vi "Over Voltage_test.vi"(8 "error in (no error)":errorcluster) -> (0 "error out":errorcluster)   [LabVIEW 2025]
uses:
  SubVIs/All test cluster.ctl
  SubVIs/All_enum_ctl.ctl
  SubVIs/Arduino_lamps.ctl
  SubVIs/Lamps_global.vi
  <vilib>/Utility/file.llb/Write Delimited Spreadsheet (string).vi
  <instrlib>/BK Precision 9200 Series/BK Precision 9200 Series.lvlib
  <instrlib>/Keithley 2260B/Keithley 2260B.lvlib
panel:
  in  "ESP PORT":refnum<visa-resource-name>
  out "Connected? 2":bool caption="Long Blank Button"
  out "Tick Time(s)":dbl
  out "Status":string
  in  "POWER SUPPLY":bool caption="Blank Button"
  out "Text name":string
  in  "COM PORT:":refnum<visa-resource-name>
  in  "Start/Stop":bool caption="Slide Switch"
  in  "File Path:":path
  in  "FILENAME":string
  out "Table":string[][](table)
  out "Connected?":bool caption="Long Blank Button"
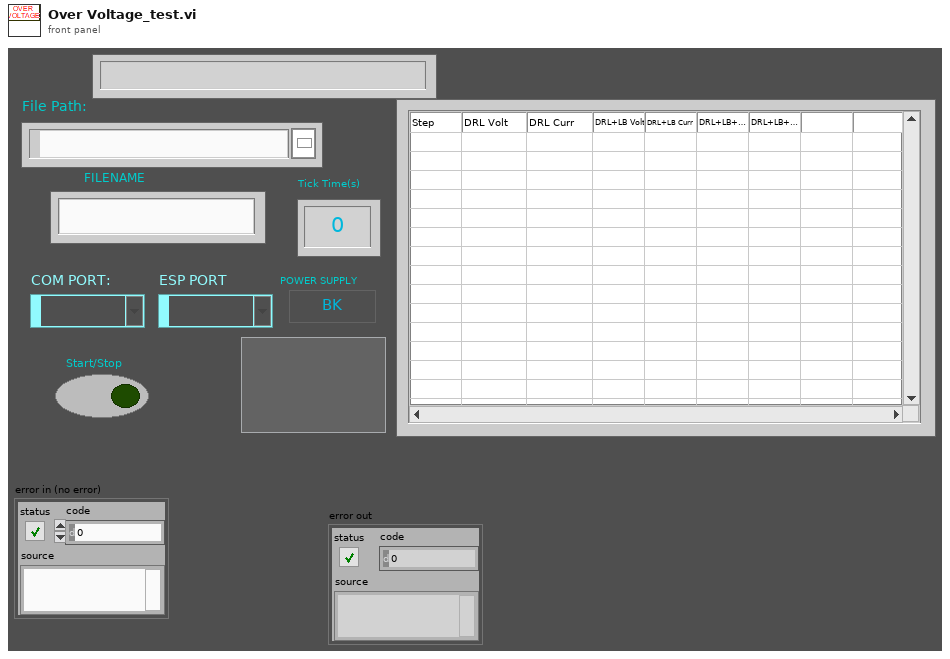
[diagram p1: front panel]
types:
  T1 = enum32{"Invalid", "Standard", "Closed", "Hidden", "Minimized", "Maximized"}
  T2 = typedef "All_enum_ctl.ctl" = enum16{"Init", "Poll", "Connect_esp32", "Connect", "check_start", "Start", "Set_Voltage", "On_relay", "Read_Voltage", "Off_Relay", "Next_Relay", "Next_Step", "Stop", "Store", "Error", "Exit"}
  T3 = typedef "All test cluster.ctl" = cluster{"FilePath":path, "Test Status":bool, "Start Volt":dbl, "End Volt":dbl, "Present Step":dbl, "Present Time(s)":dbl, "End Time":dbl, "Table":string[], "Intensity":string, "BK/Keith":bool, "COM":refnum<visa-resource-name>, "Next state":T2, "Step no.":dbl, "Start ms":u32, "ESP_COM":refnum<visa-resource-name>, "Relay_no":dbl, "Datas":string[]}
  T4 = typedef "Arduino_lamps.ctl" = enum16{"Init", "Poll", "Read", "Write", "Exit"}
  T5 = cluster{"Baud Rate":u32, "Parity":u16, "Data Bits":u16, "Stop Bits":u16, "Flow Control":u16}
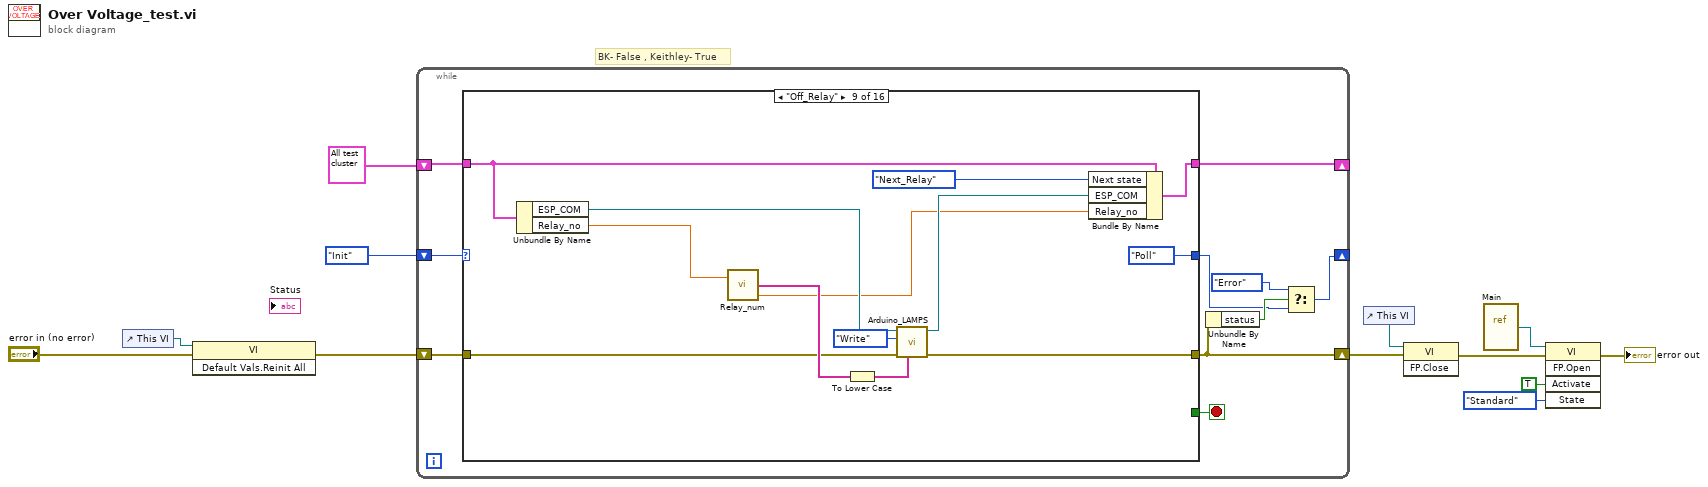
[diagram p0: block diagram]
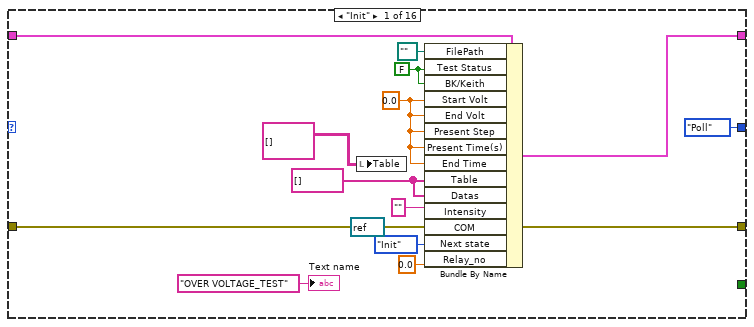
[diagram p2: hidden frame]
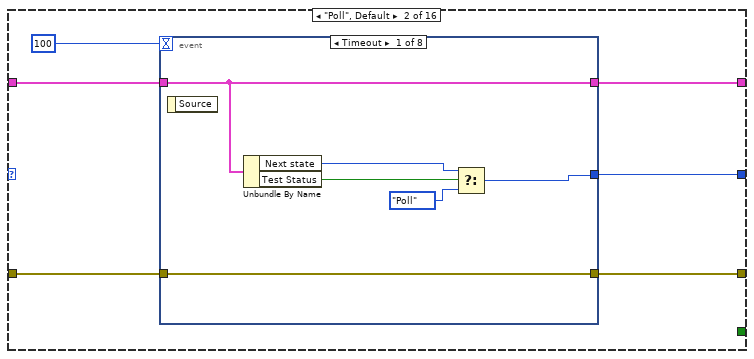
[diagram p3: hidden frame]
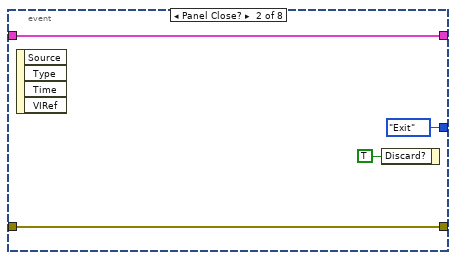
[diagram p4: hidden frame]
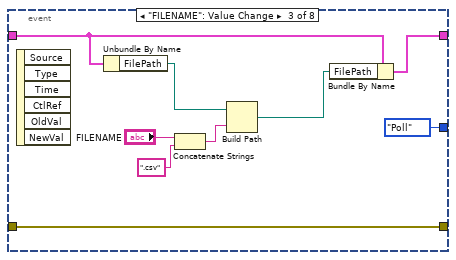
[diagram p5: hidden frame]
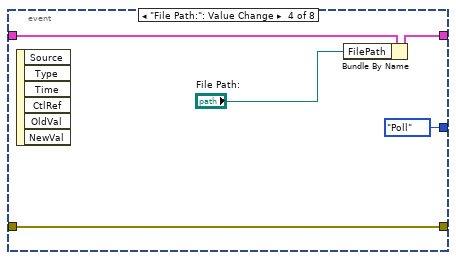
[diagram p6: hidden frame]
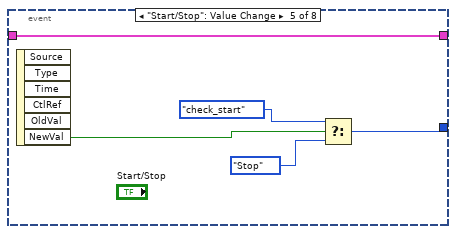
[diagram p7: hidden frame]
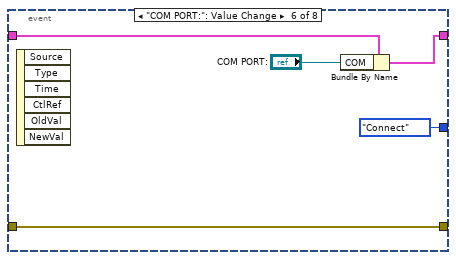
[diagram p8: hidden frame]
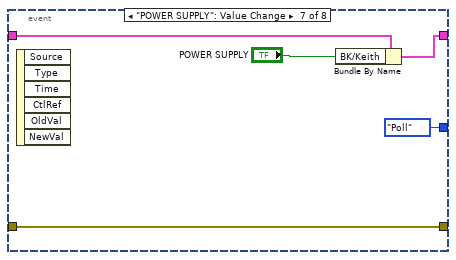
[diagram p9: hidden frame]
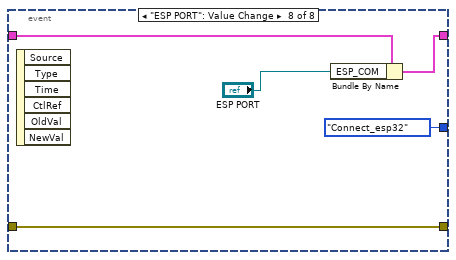
[diagram p10: hidden frame]
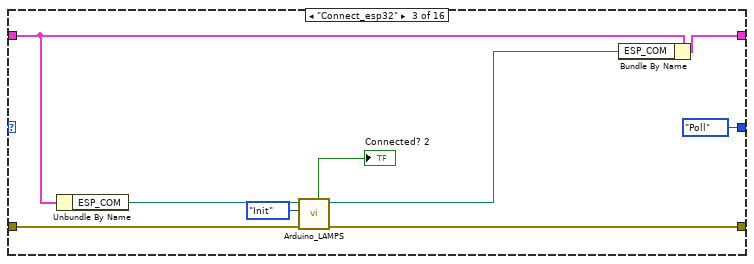
[diagram p11: hidden frame]
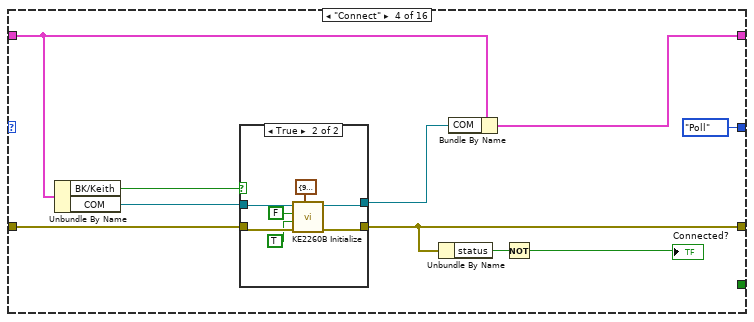
[diagram p12: hidden frame]
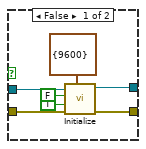
[diagram p13: hidden frame]
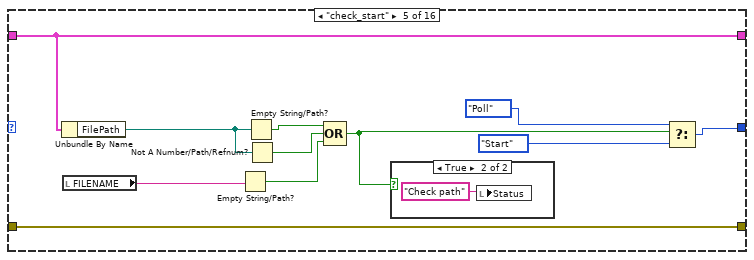
[diagram p14: hidden frame]
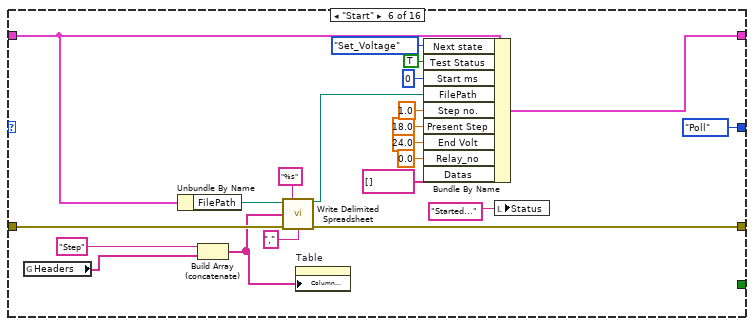
[diagram p16: hidden frame]
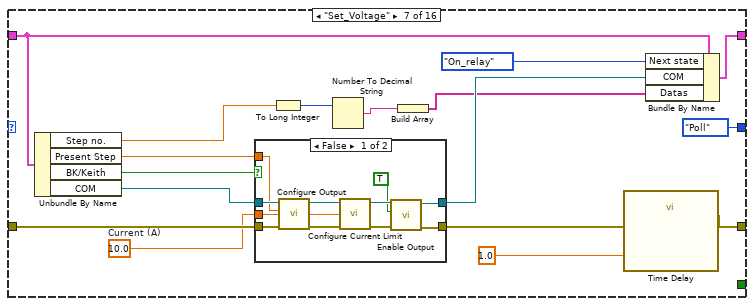
[diagram p17: hidden frame]
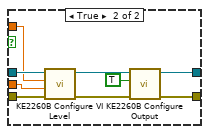
[diagram p18: hidden frame]
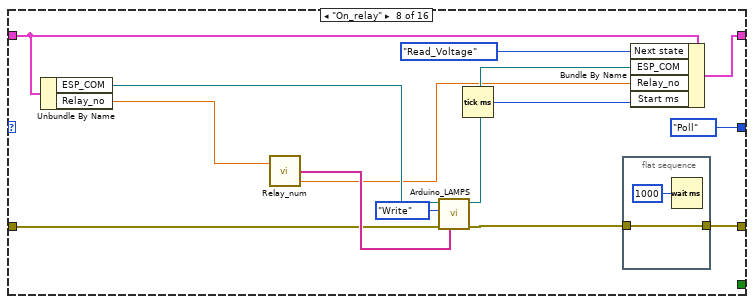
[diagram p19: hidden frame]
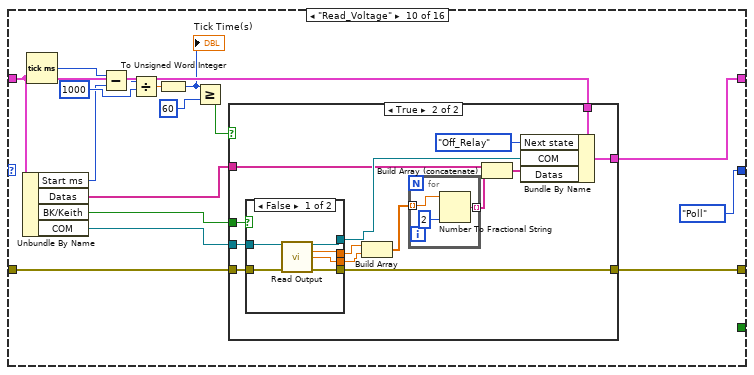
[diagram p20: hidden frame]
diagram:
  # "BK- False , Keithley- True"
  n1 = control-ref of="This VI"() -> (w12:refnum<vi>)
  n2 = invoke class="VI" method="Default Vals.Reinit All"(reference=w12, error in="error in (no error)") -> (error out=w10:errorcluster)  [unwired: 1 in, 2 out]
  n3 = while {
    shift-right: [w21] -> _
    shift-left: T3 {"FilePath"=path "", "Test Status"=FALSE, "Start Volt"=0.0, "End Volt"=0.0, "Present Step"=0.0, "Present Time(s)"=0.0, "End Time"=0.0, "Table"=[], "Intensity"="", "BK/Keith"=FALSE, "COM"="", "Next state"=enum."Init", "Step no."=0.0, "Start ms"=0, "ESP_COM"="", "Relay_no"=0.0, "Datas"=[]} -> [w20]
    shift-right: [w17] -> w2
    shift-left: w10 -> [w19]
    shift-right: [w13] -> _
    shift-left: All_enum_ctl."Init" -> [w22]
    stop <- w18 stop-if-true
    n4 = case shown="\"Off_Relay\"" w22 {
      tunnel: [w34 w39 w88 w97 w129 w151 w168 w192 w208 w229 w277 w314 w328 w342 w359 w379] -> w21
      tunnel: w20 -> [w36 w40 w91 w101 w129 w146 w167 w191 w207 w233 w278 w317 w323 w343 w362 w379]
      tunnel: w19 -> [w35 w42 w94 w105 w130 w148 w169 w195 w211 w234 w275 w318 w324 w347 w366 w384]
      tunnel: [w35 w41 w93 w100 w130 w147 w158 w194 w210 w232 w275 w311 w321 w347 w364 w380] -> w17
      tunnel: [All_enum_ctl."Poll" w37 All_enum_ctl."Poll" All_enum_ctl."Poll" w121 All_enum_ctl."Poll" All_enum_ctl."Poll" All_enum_ctl."Poll" All_enum_ctl."Poll" All_enum_ctl."Poll" All_enum_ctl."Poll" All_enum_ctl."Poll" All_enum_ctl."Poll" All_enum_ctl."Poll" All_enum_ctl."Poll" All_enum_ctl."Exit"] -> w14
      tunnel: [_ _ _ _ _ _ _ _ _ _ _ _ _ _ _ TRUE] -> w18
      frame "Init" {
        w24 = string[] [] ("Table")
        w32 = 0.0 ("Start Volt")
        w30 = FALSE ("Test Status")
        n5 = local write "Table"(string[][] [] ("Table")) -> ()
        n6 = Bundle By Name(cluster=w36, "FilePath"=path "", "Test Status"=w30, "BK/Keith"=w30, "Start Volt"=w32, "End Volt"=w32, "Present Step"=w32, "Present Time(s)"=w32, "End Time"=w32, "Table"=w24, "Datas"=w24, "Intensity"="", "COM"=refnum<visa-resource-name> refnum, "Next state"=All_enum_ctl."Init" ("Last state"), "Relay_no"=0.0) -> (w34:T3)
        "Text name" <- "OVER VOLTAGE_TEST" ("Text name")
      }
      frame "Poll", Default {
        n7 = event shown="[0] Timeout" {
          selector: _ -> [_ _ _ _ _ _ _ _]
          dyn-events: _ -> [_ _ _ _ _ _ _ _]
          timeout: 100 -> [_ _ _ _ _ _ _ _]
          tunnel: w42 -> [w48 w49 w61 w64 _ w72 w77 w82]
          tunnel: [w48 w49 w61 w64 _ w72 w77 w82] -> w41
          tunnel: w40 -> [w47 w50 w59 w66 w70 w76 w81 w85]
          tunnel: [w47 w50 w55 w63 w70 w75 w80 w86] -> w39
          tunnel: [w43 All_enum_ctl."Exit" ("f") All_enum_ctl."Poll" All_enum_ctl."Poll" w67 All_enum_ctl."Connect" ("f") All_enum_ctl."Poll" ("f") All_enum_ctl."Connect_esp32" ("f")] -> w37
          event Timeout {
            n8 = event-data() -> ()  [unwired: 1 in, 1 out]
            n9 = Unbundle By Name(w47) -> ("Next state"=w44:T2, "Test Status"=w46:bool)
            n10 = Select(t=w44, s=w46, f=All_enum_ctl."Poll") -> (s? t:f=w43:T2)
          }
          event Panel Close? {
            n11 = event-data() -> ()  [unwired: 1 in, 4 out]
            n12 = event-data("Discard?"=TRUE) -> ()  [unwired: 1 in, 1 out]
          }
          event "FILENAME": Value Change {
            n13 = event-data() -> ()  [unwired: 1 in, 6 out]
            n14 = Unbundle By Name(w59) -> ("FilePath"=w58:path)
            n15 = Concatenate Strings("FILENAME", ".csv" ("string")) -> (w57:string)
            n16 = Build Path(base path=w58, name or relative path=w57) -> (appended path=w54:path)
            n17 = Bundle By Name(cluster=w59, "FilePath"=w54) -> (w55:T3)
          }
          event "File Path:": Value Change {
            n18 = event-data() -> ()  [unwired: 1 in, 6 out]
            n19 = Bundle By Name(cluster=w66, "FilePath"="File Path:") -> (w63:T3)
          }
          event "Start/Stop": Value Change {
            n20 = event-data() -> ("NewVal"=w71:bool)  [unwired: 1 in, 5 out]
            n21 = Select(t=All_enum_ctl."check_start", s=w71, f=All_enum_ctl."Stop") -> (s? t:f=w67:T2)
          }
          event "COM PORT:": Value Change {
            n22 = event-data() -> ()  [unwired: 1 in, 6 out]
            n23 = Bundle By Name(cluster=w76, "COM"="COM PORT:") -> (w75:T3)
          }
          event "POWER SUPPLY": Value Change {
            n24 = event-data() -> ()  [unwired: 1 in, 6 out]
            n25 = Bundle By Name(cluster=w81, "BK/Keith"="POWER SUPPLY") -> (w80:T3)
          }
          event "ESP PORT": Value Change {
            n26 = event-data() -> ()  [unwired: 1 in, 6 out]
            n27 = Bundle By Name(cluster=w85, "ESP_COM"="ESP PORT") -> (w86:T3)
          }
        }
      }
      frame "Connect_esp32" {
        n28 = Unbundle By Name(w91) -> ("ESP_COM"=w90:refnum<visa-resource-name>)
        n29 = call "Arduino_LAMPS.vi"("error out"=w94, "Enum"=Arduino_lamps."Init", "VISA resource name"=w90) -> ("error out 2"=w93:errorcluster, "VISA out"=w87:refnum<visa-resource-name>, "status"=→"Connected? 2":bool)  [unwired: 4 in, 2 out]
        n30 = Bundle By Name(cluster=w91, "ESP_COM"=w87) -> (w88:T3)
      }
      frame "Connect" {
        n31 = Unbundle By Name(w101) -> ("BK/Keith"=w99:bool, "COM"=w98:refnum<visa-resource-name>)
        n32 = case shown="True" w99 {
          tunnel: w105 -> [w112 w119]
          tunnel: [w111 w118] -> w100
          tunnel: w98 -> [w110 w117]
          tunnel: [w106 w115] -> w96
          frame False {
            n33 = call <instrlib>:"Initialize.vi"("Serial Configuration"=cluster{"Baud Rate":u32} {"Baud Rate"=9600}, "error in (no error)"=w112, "Reset (True)"=TRUE, "ID Query (True)"=FALSE, "VISA resource name"=w110) -> ("error out"=w111:errorcluster, "VISA resource name out"=w106:refnum<visa-resource-name>)  [unwired: 5 in]
          }
          frame True {
            n34 = call <instrlib>:"KE2260B Initialize.vi"("Serial Configuration"=T5 {"Baud Rate"=9600, "Parity"=0, "Data Bits"=8, "Stop Bits"=10, "Flow Control"=0}, "error in (no error)"=w119, "Reset (True)"=TRUE, "ID Query (True)"=FALSE, "VISA resource name"=w117) -> ("error out"=w118:errorcluster, "VISA resource name out"=w115:refnum<visa-resource-name>)  [unwired: 5 in]
          }
        }
        n35 = Unbundle By Name(w100) -> ("status"=w104:bool)
        n36 = Bundle By Name(cluster=w101, "COM"=w96) -> (w97:T3)
        n37 = Not(x=w104) -> (.not. x?=→"Connected?":bool)
      }
      frame "check_start" {
        n38 = Unbundle By Name(w129) -> ("FilePath"=w127:path)
        n39 = local read "FILENAME"() -> (w128:string)
        n40 = Empty String/Path?(string/path=w128) -> (empty?=w124:bool)
        n41 = Empty String/Path?(string/path=w127) -> (empty?=w126:bool)
        n42 = Not A Number/Path/Refnum?(number/path/refnum=w127) -> (NaN/Path/Refnum?=w125:bool)
        n43 = Compound Arithmetic op=OR(w126, w125, w124) -> (w120:bool)
        n44 = case shown="True" w120 {
          frame False {
          }
          frame True {
            n45 = local write "Status"("Check path") -> ()
          }
        }
        n46 = Select(t=All_enum_ctl."Poll", s=w120, f=All_enum_ctl."Start") -> (s? t:f=w121:T2)
      }
      frame "Start" {
        n47 = global read "Lamps_global.vi" "Headers"() -> (w134:string[])
        n48 = Unbundle By Name(w146) -> ("FilePath"=w145:path)
        n49 = Build Array (concatenate)("Step" ("String"), w134) -> (w133:string[])
        n50 = call-poly <vilib>:"Write Delimited Spreadsheet.vi"("file path (dialog if empty)"=w145, "format (%s)"="%s" ("format (%.3f)"), "1D data"=w133, "error in (no error)"=w148, "delimiter (\\t)"="," ("delimiter (\\t)")) -> ("new file path (Not A Path if cancelled)"=w142:path, "error out"=w147:errorcluster)  [unwired: 9 in]
        n51 = property on="Table" class="Tbl (strict)"("Column Headers[]"=w133) -> ()  [unwired: 2 in, 2 out]
        n52 = Bundle By Name(cluster=w146, "Next state"=All_enum_ctl."Set_Voltage" ("Last state"), "Test Status"=TRUE, "Start ms"=u32 0, "FilePath"=w142, "Step no."=1.0, "Present Step"=18.0, "End Volt"=24.0, "Relay_no"=0.0, "Datas"=string[] []) -> (w151:T3)
        n53 = local write "Status"("Started...") -> ()
      }
      frame "Set_Voltage" {
        w160 = 10.0  # Current (A)
        n54 = Unbundle By Name(w167) -> ("Step no."=w154:dbl, "Present Step"=w161:dbl, "BK/Keith"=w162:bool, "COM"=w165:refnum<visa-resource-name>)
        n55 = case shown="False" w162 {
          tunnel: w169 -> [w173 w189]
          tunnel: [w180 w188] -> w166
          tunnel: w165 -> [w178 w186]
          tunnel: [w179 w184] -> w164
          tunnel: w161 -> [w177 w182]
          tunnel: w160 -> [w171 w181]
          frame False {
            n56 = call <instrlib>:"Configure Output.vi"("error in (no error)"=w173, "Voltage Level (0.0 V)"=w177, "VISA resource name"=w178) -> ("error out"=w174:errorcluster, "VISA resource name out"=w172:refnum<visa-resource-name>)  [unwired: 7 in]
            n57 = call <instrlib>:"Configure Current Limit.vi"("error in (no error)"=w174, "Current Limit (0.0 A)"=w171, "VISA resource name"=w172) -> ("error out"=w176:errorcluster, "VISA resource name out"=w175:refnum<visa-resource-name>)  [unwired: 7 in]
            n58 = call <instrlib>:"Enable Output.vi"("error in (no error)"=w176, "Enable Output (F: False)"=TRUE, "VISA resource name"=w175) -> ("error out"=w180:errorcluster, "VISA resource name out"=w179:refnum<visa-resource-name>)  [unwired: 7 in]
          }
          frame True {
            n59 = call <instrlib>:"KE2260B Configure VI Level.vi"("error in (no error)"=w189, "Current Level (0.000 A)"=w181, "Voltage Level (0.000 V)"=w182, "VISA resource name"=w186) -> ("error out"=w187:errorcluster, "VISA resource name out"=w185:refnum<visa-resource-name>)  [unwired: 6 in]
            n60 = call <instrlib>:"KE2260B Configure Output.vi"("error in (no error)"=w187, "Enable Output (T: Enable)"=TRUE, "VISA resource name"=w185) -> ("error out"=w188:errorcluster, "VISA resource name out"=w184:refnum<visa-resource-name>)  [unwired: 7 in]
          }
        }
        n61 = To Long Integer(number=w154) -> (32bit integer=w156:i32)
        n62 = Number To Decimal String(number=w156) -> (decimal integer string=w155:string)  [unwired: 1 in]
        n63 = Build Array(w155) -> (w153:string[])
        n64 = call "Time Delay"("error in (no error)"=w166, "Delay Time (s)"=1.0) -> ("error out"=w158:errorcluster)  [unwired: 9 in]
        n65 = Bundle By Name(cluster=w167, "Next state"=All_enum_ctl."On_relay", "COM"=w164, "Datas"=w153) -> (w168:T3)
      }
      frame "On_relay" {
        n66 = Unbundle By Name(w191) -> ("ESP_COM"=w203:refnum<visa-resource-name>, "Relay_no"=w198:dbl)
        n67 = call "Relay_num.vi"("Relay_no."=w198) -> ("Relay"=w197:string[], "Relay_no.out"=w196:dbl)  [unwired: 1 in, 1 out]
        n68 = call "Arduino_LAMPS.vi"("DO's"=w197, "error out"=w195, "Enum"=Arduino_lamps."Write", "VISA resource name"=w203) -> ("error out 2"=w199:errorcluster, "VISA out"=w201:refnum<visa-resource-name>)  [unwired: 3 in, 3 out]
        n69 = Tick Count (ms)() -> (millisecond timer value=w190:u32)
        n70 = flat-sequence {
          tunnel: w199 -> [w205]
          tunnel: [w205] -> w194
          frame #0 {
            n71 = Wait (ms)(milliseconds to wait=u32 1000) -> ()  [unwired: 1 out]
          }
        }
        n72 = Bundle By Name(cluster=w191, "Next state"=All_enum_ctl."Read_Voltage", "ESP_COM"=w201, "Relay_no"=w196, "Start ms"=w190) -> (w192:T3)
      }
      frame "Off_Relay" {
        n73 = Unbundle By Name(w207) -> ("ESP_COM"=w218:refnum<visa-resource-name>, "Relay_no"=w214:dbl)
        n74 = call "Relay_num.vi"("Relay_no."=w214) -> ("Relay"=w213:string[], "Relay_no.out"=w212:dbl)  [unwired: 1 in, 1 out]
        n75 = To Lower Case(string=w213) -> (all lower case string=w206:string[])
        n76 = call "Arduino_LAMPS.vi"("DO's"=w206, "error out"=w211, "Enum"=Arduino_lamps."Write", "VISA resource name"=w218) -> ("error out 2"=w210:errorcluster, "VISA out"=w216:refnum<visa-resource-name>)  [unwired: 3 in, 3 out]
        n77 = Bundle By Name(cluster=w207, "Next state"=All_enum_ctl."Next_Relay", "ESP_COM"=w216, "Relay_no"=w212) -> (w208:T3)
      }
      frame "Read_Voltage" {
        n78 = Unbundle By Name(w233) -> ("Start ms"=w219:u32, "Datas"=w227:string[], "BK/Keith"=w230:bool, "COM"=w231:refnum<visa-resource-name>)
        n79 = Tick Count (ms)() -> (millisecond timer value=w224:u32)
        n80 = Subtract(x=w224, y=w219) -> (x-y=w226:u32)
        n81 = Divide(x=w226, y=u32 1000) -> (x/y=w225:dbl)
        n82 = To Unsigned Word Integer(number=w225) -> (unsigned 16bit integer=w223:u16)
        "Tick Time(s)" <- w223
        n83 = Greater Or Equal?(x=w223, y=u16 60) -> (x >= y?=w220:bool)
        n84 = case shown="True" w220 {
          tunnel: w234 -> [w239 w257]
          tunnel: w233 -> [w235 w256]
          tunnel: [w238 w255] -> w232
          tunnel: w231 -> [_ w254]
          tunnel: w230 -> [_ w253]
          tunnel: [w235 w252] -> w229
          tunnel: w227 -> [_ w244]
          frame False {
            n85 = flat-sequence {
              tunnel: w239 -> [w241]
              tunnel: [w241] -> w237
              tunnel: [u32 1000 ("milliseconds to wait")] -> w236
              tunnel: [w243] -> w238
              tunnel: w237 -> [w243]
              tunnel: w236 -> [w242]
              frame #0 {
              }
              frame #1 {
                n86 = Wait (ms)(milliseconds to wait=w242) -> ()  [unwired: 1 out]
              }
            }
          }
          frame True {
            n87 = case shown="False" w253 {
              tunnel: w257 -> [w263 w269]
              tunnel: [w262 w268] -> w255
              tunnel: w254 -> [w261 w266]
              tunnel: [w260 w267] -> w251
              tunnel: [w259 w265] -> w249
              tunnel: [w258 w264] -> w248
              frame False {
                n88 = call <instrlib>:"Read Output.vi"("VISA resource name"=w261, "error in (no error)"=w263) -> ("VISA resource name out"=w260:refnum<visa-resource-name>, "Actual Voltage Level (V)"=w259:dbl, "Actual Current Level (A)"=w258:dbl, "error out"=w262:errorcluster)  [unwired: 9 in, 1 out]
              }
              frame True {
                n89 = call <instrlib>:"KE2260B Read Output.vi"("error in (no error)"=w269, "VISA resource name"=w266) -> ("error out"=w268:errorcluster, "Actual Current Level (A)"=w264:dbl, "Actual Voltage Level (V)"=w265:dbl, "VISA resource name out"=w267:refnum<visa-resource-name>)  [unwired: 6 in]
              }
            }
            n90 = Build Array(w249, w248) -> (w247:dbl[])
            n91 = for {
              tunnel: w247 -> [w271] mode=indexing
              tunnel: [w270] -> w246 mode=indexing
              n92 = Number To Fractional String(number=w271, precision (6)=i16 2) -> (F-format string=w270:string)  [unwired: 2 in]
            }
            n93 = Build Array (concatenate)(w244, w246) -> (w245:string[])
            n94 = Bundle By Name(cluster=w256, "Next state"=All_enum_ctl."Off_Relay", "COM"=w251, "Datas"=w245) -> (w252:T3)
          }
        }
      }
      frame "Next_Relay" {
        n95 = property on="Table" class="Tbl (strict)"() -> ("Column Headers[]"=w274:string[])  [unwired: 2 in, 2 out]
        n96 = Unbundle By Name(w278) -> ("Relay_no"=w282:dbl, "Datas"=w279:string[])
        n97 = Array Size(array=w274) -> (size(s)=w273:i32)
        n98 = call "Relay_num.vi"("Relay_no."=w282) -> ("x = y?"=w281:bool, "Relay_no.out"=w280:dbl)  [unwired: 1 in, 1 out]
        n99 = case shown="False" w281 {
          tunnel: [w298 w303] -> w277
          tunnel: w278 -> [w297 w302]
          tunnel: w280 -> [w295 _]
          tunnel: w279 -> [w287 w299]
          tunnel: w273 -> [w288 _]
          frame False {
            n100 = Increment(x=w295) -> (x+1=w294:dbl)
            n101 = local read "Table"() -> (w293:string[][])
            n102 = Array Size(array=w287) -> (size(s)=w291:i32)
            n103 = Subtract(x=w288, y=w291) -> (x-y=w290:i32)
            n104 = Array Size(array=w293) -> (size(s)=w292:i32[])
            n105 = Index Array(array=w292) -> (element=w283:i32)  [unwired: 1 in]
            n106 = Initialize Array("", w290) -> (w289:string[])
            n107 = Build Array (concatenate)(w287, w289) -> (w285:string[])
            n108 = Replace Array Subset(array=w293, new element=w285, index (row)=w283) -> (w284:string[][])  [unwired: 1 in]
            n109 = property on="Table" class="Tbl (strict)"("Value"=w284) -> ()  [unwired: 2 in, 2 out]
            n110 = Bundle By Name(cluster=w297, "Next state"=All_enum_ctl."On_relay", "Relay_no"=w294, "Datas"=w287) -> (w298:T3)
          }
          frame True {
            n111 = Bundle By Name(cluster=w302, "Next state"=All_enum_ctl."Store", "Relay_no"=0.0, "Table"=w299) -> (w303:T3)
          }
        }
      }
      frame "Store" {
        n112 = Unbundle By Name(w317) -> ("Table"=w308:string[], "FilePath"=w310:path)
        n113 = local read "Table"() -> (w316:string[][])
        n114 = Build Array (concatenate)(w316, w308) -> (→"Table":string[][])
        n115 = call-poly <vilib>:"Write Delimited Spreadsheet.vi"("file path (dialog if empty)"=w310, "format (%s)"="%s", "1D data"=w308, "append to file? (new file:F)"=TRUE, "error in (no error)"=w318, "delimiter (\\t)"="," ("delimiter (\\t)")) -> ("new file path (Not A Path if cancelled)"=w307:path, "error out"=w311:errorcluster)  [unwired: 8 in]
        n116 = Bundle By Name(cluster=w317, "Next state"=All_enum_ctl."Next_Step", "FilePath"=w307, "Datas"=string[] []) -> (w314:T3)
      }
      frame "Stop" {
        n117 = Unbundle By Name(w323) -> ("BK/Keith"=w325:bool, "COM"=w326:refnum<visa-resource-name>)
        n118 = case shown="False" w325 {
          tunnel: w324 -> [w332 w338]
          tunnel: [w334 w339] -> w321
          tunnel: w326 -> [w331 w337]
          tunnel: [w333 w336] -> w322
          frame False {
            n119 = call <instrlib>:"Enable Output.vi"("error in (no error)"=w332, "Enable Output (F: False)"=FALSE, "VISA resource name"=w331) -> ("error out"=w334:errorcluster, "VISA resource name out"=w333:refnum<visa-resource-name>)  [unwired: 7 in]
          }
          frame True {
            n120 = call <instrlib>:"KE2260B Configure Output.vi"("error in (no error)"=w338, "Enable Output (T: Enable)"=FALSE, "VISA resource name"=w337) -> ("error out"=w339:errorcluster, "VISA resource name out"=w336:refnum<visa-resource-name>)  [unwired: 7 in]
          }
        }
        n121 = local write "Start/Stop"(FALSE ("Start/Stop")) -> ()
        n122 = Bundle By Name(cluster=w323, "Test Status"=FALSE, "COM"=w322) -> (w328:T3)
        n123 = local write "Status"("Test Stopped....") -> ()
      }
      frame "Next_Step" {
        n124 = Unbundle By Name(w343) -> ("Present Step"=w344:dbl, "End Volt"=w345:dbl, "Step no."=w340:dbl)
        n125 = Equal?(x=w344, y=w345) -> (x = y?=w346:bool)
        n126 = case shown="False" w346 {
          tunnel: w344 -> [_ _]
          tunnel: w343 -> [w354 w357]
          tunnel: [w353 w356] -> w342
          tunnel: w340 -> [w351 _]
          frame False {
            n127 = Increment(x=w351) -> (x+1=w350:dbl)
            n128 = Tick Count (ms)() -> (millisecond timer value=w348:u32)
            n129 = Bundle By Name(cluster=w354, "Start ms"=w348, "Next state"=All_enum_ctl."Set_Voltage", "Present Step"=24.0, "Step no."=w350) -> (w353:T3)
          }
          frame True {
            n130 = Bundle By Name(cluster=w357, "Next state"=All_enum_ctl."Stop") -> (w356:T3)
          }
        }
      }
      frame "Error" {
        n131 = Unbundle By Name(w362) -> ("BK/Keith"=w360:bool, "COM"=w361:refnum<visa-resource-name>)
        n132 = case shown="False" w360 {
          tunnel: w366 -> [w369 w374]
          tunnel: [w370 w373] -> w363
          tunnel: w361 -> [w368 w372]
          tunnel: [w367 w371] -> w358
          frame False {
            n133 = call <instrlib>:"Reset.vi"("error in (no error)"=w369, "VISA resource name"=w368) -> ("error out"=w370:errorcluster, "VISA resource name out"=w367:refnum<visa-resource-name>)  [unwired: 8 in]
          }
          frame True {
            n134 = call <instrlib>:"KE2260B Reset.vi"("error in (no error)"=w374, "VISA resource name"=w372) -> ("error out"=w373:errorcluster, "VISA resource name out"=w371:refnum<visa-resource-name>)  [unwired: 8 in]
          }
        }
        n135 = call <vilib>:"Clear Errors.vi"("error in (no error)"=w363) -> ("error out"=w364:errorcluster)  [unwired: 5 in, 1 out]
        n136 = Bundle By Name(cluster=w362, "COM"=w358) -> (w359:T3)
      }
      frame "Exit" {
        n137 = Unbundle By Name(w379) -> ("ESP_COM"=w375:refnum<visa-resource-name>, "BK/Keith"=w377:bool, "COM"=w378:refnum<visa-resource-name>)
        n138 = case shown="False" w377 {
          tunnel: w384 -> [w387 w390]
          tunnel: [w386 w389] -> w381
          tunnel: w378 -> [w385 w388]
          frame False {
            n139 = call <instrlib>:"Close.vi"("error in (no error)"=w387, "VISA resource name"=w385) -> ("error out"=w386:errorcluster)  [unwired: 9 in]
          }
          frame True {
            n140 = call <instrlib>:"KE2260B Close.vi"("error in (no error)"=w390, "VISA resource name"=w388) -> ("error out"=w389:errorcluster)  [unwired: 9 in]
          }
        }
        n141 = VISA Close(VISA resource name=w375, error in (no error)=w381) -> (error out=w376:errorcluster)
        n142 = call <vilib>:"Clear Errors.vi"("error in (no error)"=w376) -> ("error out"=w380:errorcluster)  [unwired: 5 in, 1 out]
      }
    }
    n143 = Unbundle By Name(w17) -> ("status"=w16:bool)
    n144 = Select(t=All_enum_ctl."Error", s=w16, f=w14) -> (s? t:f=w13:T2)
  }
  n145 = control-ref of="This VI"() -> (w3:refnum<vi>)
  n146 = invoke class="VI" method="FP.Close"(reference=w3, error in=w2) -> (error out=w1:errorcluster)  [unwired: 1 in, 2 out]
  n147 = vi-ref "Main.vi"() -> (w7:refnum<vi>)
  n148 = invoke class="VI" method="FP.Open"(reference=w7, error in=w1, "Activate"=TRUE ("Activate?"), "State"=T1."Standard") -> (error out=→"error out":errorcluster)  [unwired: 1 in, 4 out]
